vi "Inspect_Pins.vi"(6 "Pitch Tol (mm)":dbl, 9 "Expected Pin Count":i32, 10 "Nominal Pitch (mm)":dbl, 11 "Image":u8[][](array[numeric])) -> (0 "Pins OK":bool, 1 "Max Pitch Dev (mm)":dbl, 2 "Pitch (mm)":dbl[](array[numeric]), 3 "Pin Centers (px)":dbl[](array[numeric]), 4 "Defect":string, 5 "Pin Count":i32, 7 "Profile":dbl[](graph))   [LabVIEW 2018]
uses:
  <vilib>/Analysis/NI_AALBase.lvlib
  <vilib>/Analysis/baseanly.llb/Mean (DBL).vi
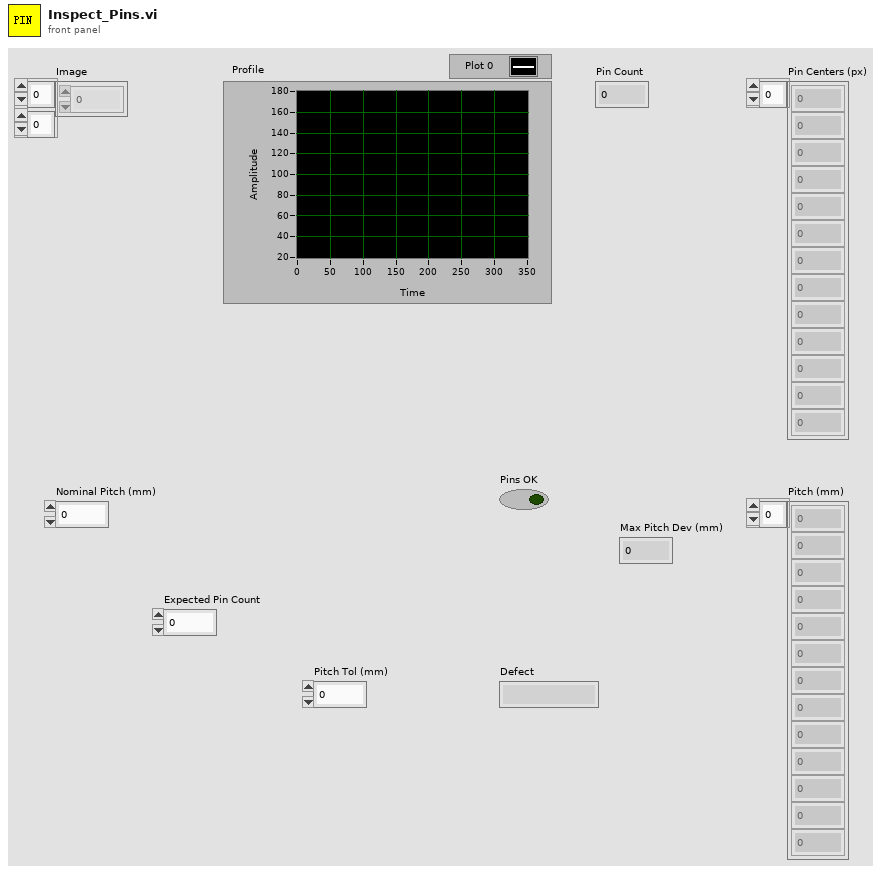
[diagram p1: front panel]
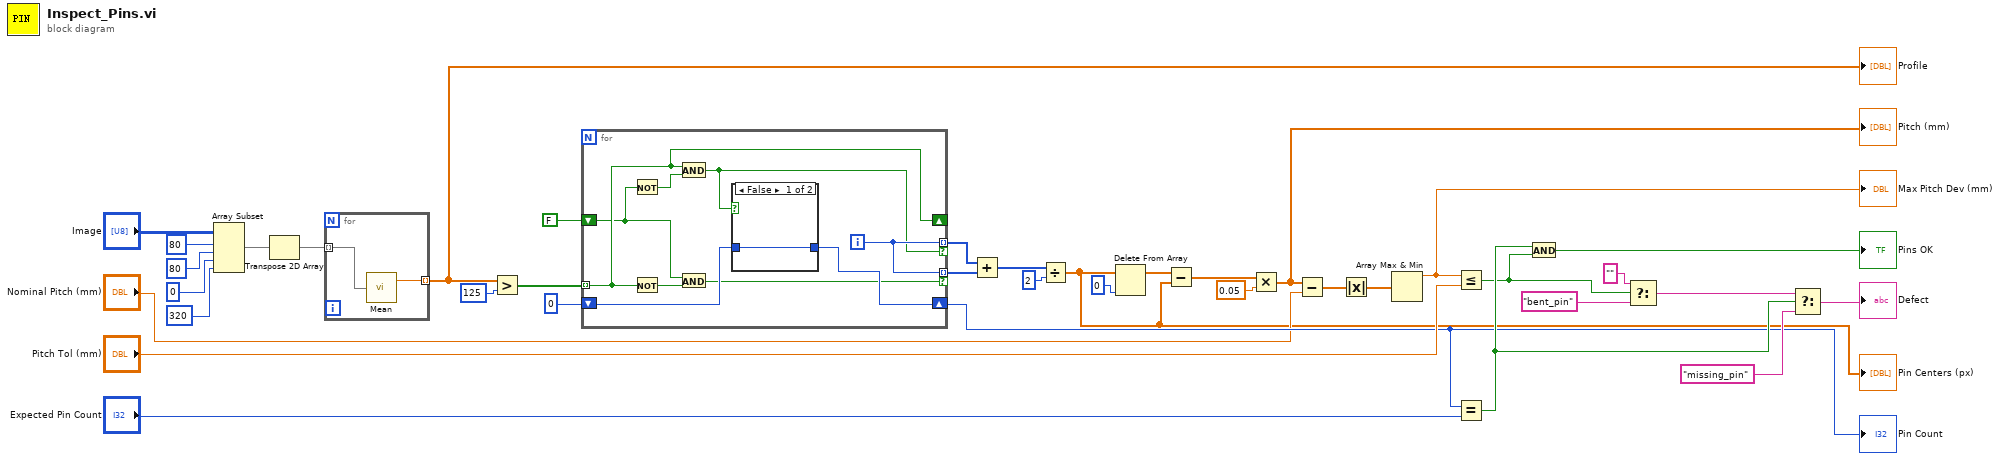
[diagram p0: block diagram]
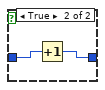
[diagram p2: hidden frame]
diagram:
  n1 = Array Subset(array="Image", index (row)=80 ("index"), length (row)=80 ("length"), index (col)=0 ("index"), length (col)=320 ("length")) -> (w6:u8[][])
  n2 = Transpose 2D Array(2D array=w6) -> (transposed array=w7:u8[][])
  n3 = for {
    tunnel: w7 -> [w39] mode=indexing
    tunnel: [w38] -> w8 mode=indexing
    n4 = call-poly <vilib>:"Mean.vi"("X"=w39) -> ("mean"=w38:dbl)  [unwired: 1 out]
  }
  "Profile" <- w8
  n5 = Greater?(x=w8, y=125) -> (0:w10:bool[])
  n6 = for {
    tunnel: w10 -> [w45] mode=indexing
    shift-right: [w46] -> w26
    shift-left: 0 -> [w47]
    shift-right: [w45] -> _
    shift-left: FALSE -> [w44]
    tunnel: [w42] -> w14 mode=indexing if=w40
    tunnel: [w42] -> w13 mode=indexing if=w41
    i -> [w42]
    n7 = Not(x=w44) -> (.not. x?=w48:bool)
    n8 = Not(x=w45) -> (.not. x?=w43:bool)
    n9 = And(x=w45, y=w48) -> (x .and. y?=w41:bool)
    n10 = And(x=w44, y=w43) -> (x .and. y?=w40:bool)
    n11 = case shown="False" w41 {
      tunnel: w47 -> [w49 w51]
      tunnel: [w49 w50] -> w46
      frame False {
      }
      frame True {
        n12 = Increment(x=w51) -> (x+1=w50:i32)
      }
    }
  }
  "Pin Count" <- w26
  n13 = Add(x=w13, y=w14) -> (x+y=w15:i32[])
  n14 = Divide(x=w15, y=2) -> (x/y=w19:dbl[])
  "Pin Centers (px)" <- w19
  n15 = Delete From Array(array=w19, index=0) -> (array with subset deleted=w18:dbl[])  [unwired: 1 in, 1 out]
  n16 = Subtract(x=w18, y=w19) -> (x-y=w20:dbl[])
  n17 = Multiply(x=w20, y=0.05) -> (x*y=w22:dbl[])
  "Pitch (mm)" <- w22
  n18 = Subtract(x=w22, y="Nominal Pitch (mm)") -> (x-y=w24:dbl[])
  n19 = Absolute Value(x=w24) -> (abs(x)=w25:dbl[])
  n20 = Array Max & Min(array=w25) -> (max value=w28:dbl)  [unwired: 3 out]
  "Max Pitch Dev (mm)" <- w28
  n21 = Less Or Equal?(x=w28, y="Pitch Tol (mm)") -> (x <= y?=w31:bool)
  n22 = Equal?(x=w26, y="Expected Pin Count") -> (x = y?=w34:bool)
  n23 = And(x=w34, y=w31) -> (x .and. y?=→"Pins OK":bool)
  n24 = Select(t="", s=w31, f="bent_pin") -> (s? t:f=w35:string)
  n25 = Select(t=w35, s=w34, f="missing_pin") -> (s? t:f=→"Defect":string)
